vi "Project Lab VIew.vi"() -> ()   [LabVIEW 2026]
uses:
  <vilib>/httpClient/POSTBuffer.vi
  <vilib>/httpClient/LabVIEWHTTPClient.lvlib
panel:
  in  "stop":bool
  out "Supervisory Health Banner":string
  in  "Plant Mode":bool
  out "Web Bridge TX":bool
  out "Live Plant Trend Recorder":cluster{"upper limit":dbl, dbl, dbl}(graph)
  out "CRITICAL PLANT INTERLOCK":bool
  in  "Fan Manual Run":bool
  in  "Valve Override":bool
  out "Fan Active":bool
  out "Valve Open":bool
  in  "Pump Override":bool
  out "Pump Running":bool
  out "Pump Current (A)":dbl(knob) scale=0.0..5.0
  out "12V Bus Voltage (V)":dbl(knob) scale=0.0..20.0
  out "Gas Hazard Level (%)":dbl
  out "Thermometer":dbl(slide) scale=0.0..100.0
  out "Volume (Liters)":dbl
  out "Level (cm)":dbl
  out "Tank Level (cm)":dbl(slide) scale=0.0..100.0
  # "SIMULATION / DIGITAL TWIN"
  # "LIVE HARDWARE (ESP32)"
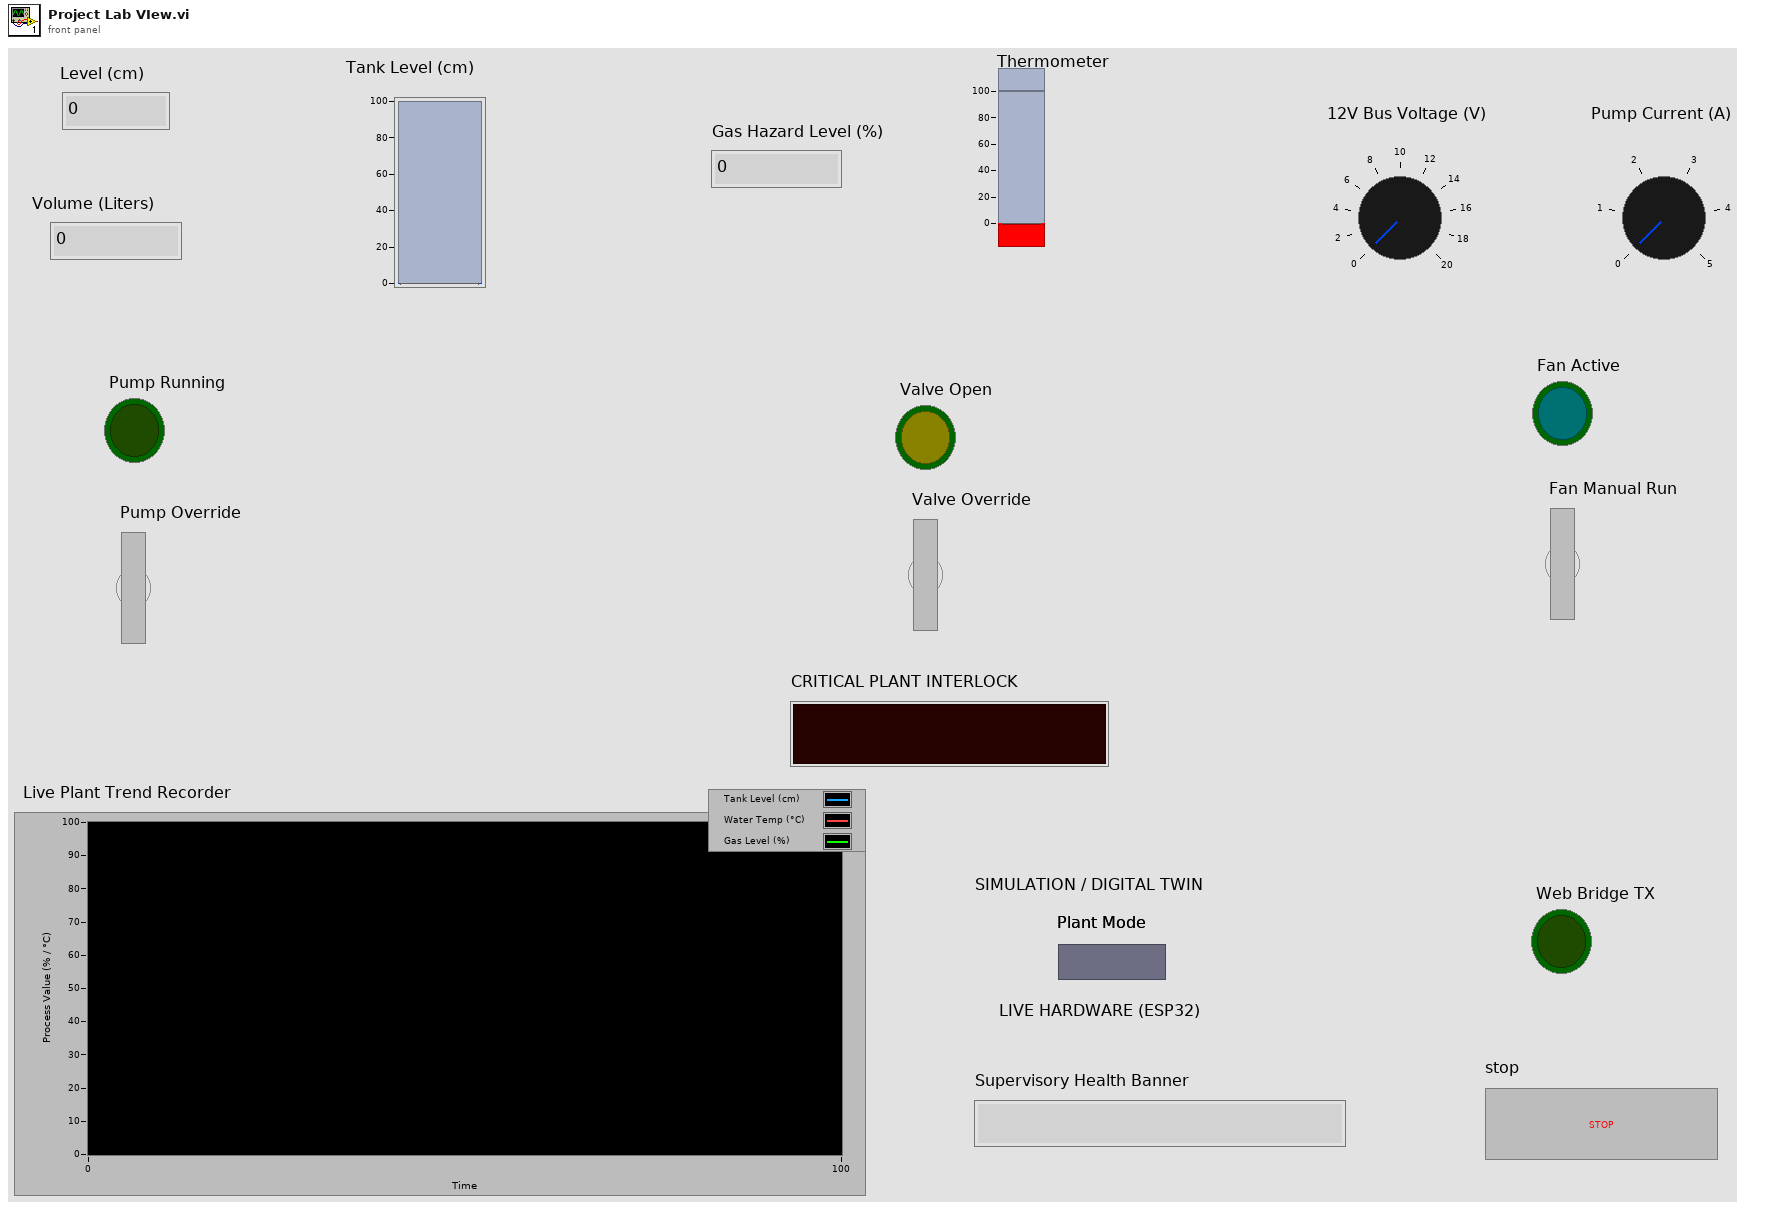
[diagram p1: front panel]
types:
  T1 = cluster{"tank_level":dbl, "temperature":dbl, "gas_ppm":dbl, "current_draw":dbl, "valve_open":bool, "fan_active":bool, "pump_active":bool}
  T2 = cluster{"water_temp_c":dbl, "gas_pct":dbl, "bus_v":dbl, "pump_a":dbl, "pump":dbl, "valve":dbl, "fan":dbl, "alarm":dbl, "level_cm":dbl}
  T3 = cluster{"upper limit":dbl, "water_temp_c":dbl, "gas_pct":dbl}
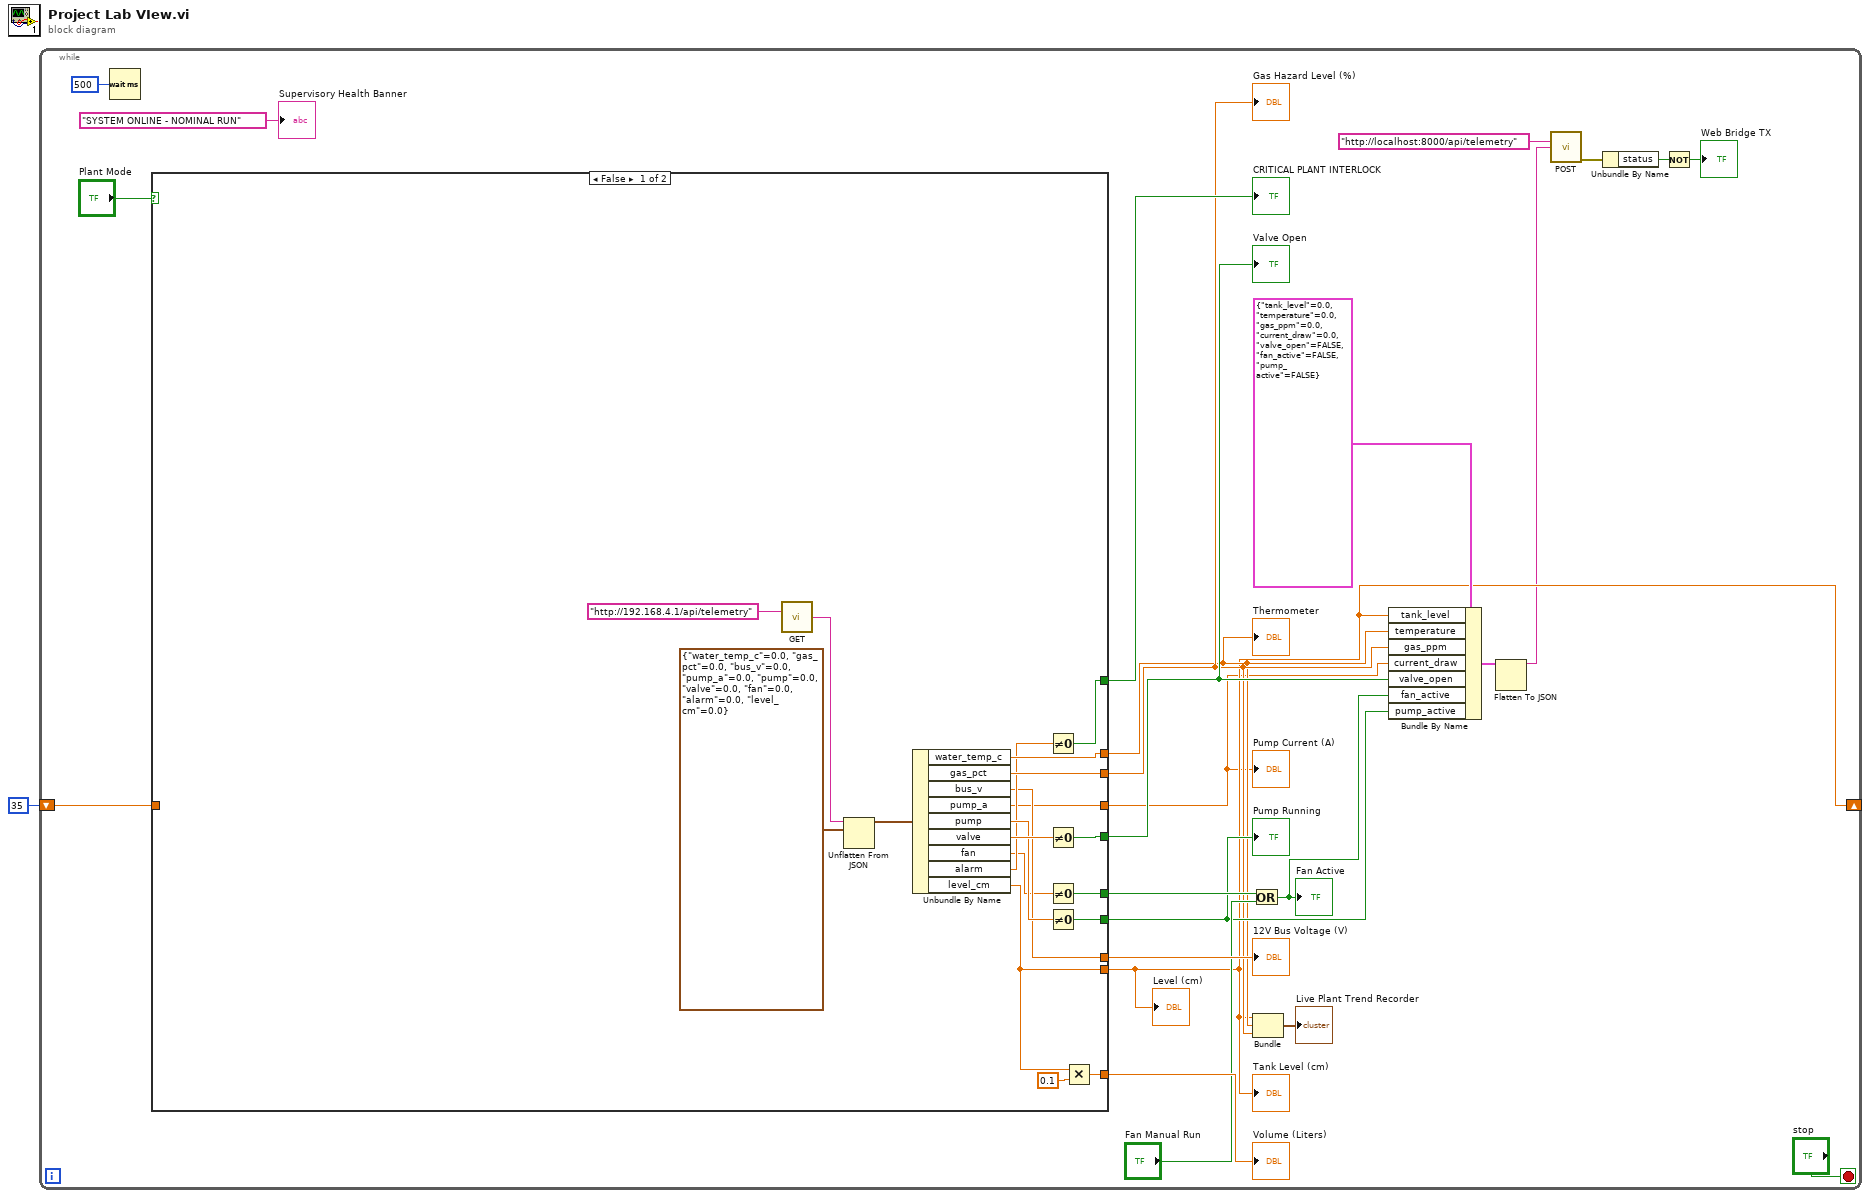
[diagram p0: block diagram]
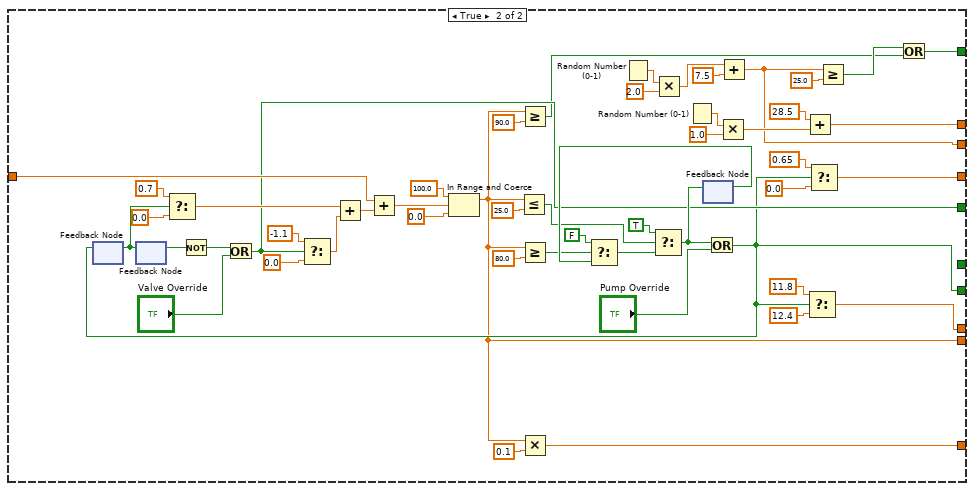
[diagram p2: hidden frame]
diagram:
  n1 = while {
    shift-right: [w9] -> _
    shift-left: u32 35 ("milliseconds to wait") -> [w24]
    stop <- "stop" stop-if-true
    n2 = Wait (ms)(milliseconds to wait=u32 500) -> ()  [unwired: 1 out]
    n3 = case shown="False" "Plant Mode" {
      tunnel: w24 -> [_ w89]
      tunnel: [w39 w52] -> w9
      tunnel: [w40 w71] -> w21
      tunnel: [w42 w66] -> w10
      tunnel: [w38 w50] -> w11
      tunnel: [w31 w58] -> w22
      tunnel: [w30 w55] -> w8
      tunnel: [w33 w53] -> w12
      tunnel: [w34 w54] -> w14
      tunnel: [w32 w46] -> w23
      tunnel: [w27 _] -> w16
      frame False {
        n4 = call <vilib>:"GET.vi"("url"="http://192.168.4.1/api/telemetry") -> ("body"=w29:string)  [unwired: 11 in, 3 out]
        n5 = Unflatten From JSON(JSON string=w29, type and defaults=T2 {"water_temp_c"=0.0, "gas_pct"=0.0, "bus_v"=0.0, "pump_a"=0.0, "pump"=0.0, "valve"=0.0, "fan"=0.0, "alarm"=0.0, "level_cm"=0.0}) -> (value=w43:T2)  [unwired: 5 in, 1 out]
        n6 = Unbundle By Name(w43) -> ("water_temp_c"=w42:dbl, "gas_pct"=w38:dbl, "bus_v"=w31:dbl, "pump_a"=w30:dbl, "pump"=w36:dbl, "valve"=w37:dbl, "fan"=w28:dbl, "alarm"=w35:dbl, "level_cm"=w39:dbl)
        n7 = Not Equal To 0?(x=w35) -> (x != 0?=w32:bool)
        n8 = Not Equal To 0?(x=w37) -> (x != 0?=w34:bool)
        n9 = Not Equal To 0?(x=w28) -> (x != 0?=w27:bool)
        n10 = Not Equal To 0?(x=w36) -> (x != 0?=w33:bool)
        n11 = Multiply(x=w39, y=0.1) -> (x*y=w40:dbl)
      }
      frame True {
        n12 = feedback #1() -> (w61:bool)  [unwired: 1 in]
        n13 = feedback-in #2(w61) -> ()
        n14 = feedback #2() -> (w73:bool)  [unwired: 1 in]
        n15 = Select(t=0.7, s=w61, f=0.0) -> (s? t:f=w92:dbl)
        n16 = Not(x=w73) -> (.not. x?=w77:bool)
        n17 = Or(x=w77, y="Valve Override") -> (x .or. y?=w54:bool)
        n18 = Select(t=-1.1, s=w54, f=0.0) -> (s? t:f=w91:dbl)
        n19 = Add(x=w92, y=w91) -> (x+y=w90:dbl)
        n20 = Add(x=w89, y=w90) -> (x+y=w86:dbl)
        n21 = In Range and Coerce(upper limit=100.0, x=w86, lower limit=0.0) -> (coerced(x)=w52:dbl)  [unwired: 1 out]
        n22 = Less Or Equal?(x=w52, y=25.0) -> (x <= y?=w75:bool)
        n23 = Greater Or Equal?(x=w52, y=90.0) -> (x >= y?=w47:bool)
        n24 = Greater Or Equal?(x=w52, y=80.0) -> (x >= y?=w74:bool)
        n25 = Multiply(x=w52, y=0.1) -> (x*y=w71:dbl)
        n26 = Random Number (0-1)() -> (number: 0 to 1=w65:dbl)
        n27 = Multiply(x=w65, y=2.0) -> (x*y=w63:dbl)
        n28 = Random Number (0-1)() -> (number: 0 to 1=w70:dbl)
        n29 = feedback #3() -> (w80:bool)  [unwired: 1 in]
        n30 = Select(t=FALSE, s=w74, f=w80) -> (s? t:f=w81:bool)
        n31 = Select(t=TRUE, s=w75, f=w81) -> (s? t:f=w78:bool)
        n32 = feedback-in #3(w78) -> ()
        n33 = Or(x=w78, y="Pump Override") -> (x .or. y?=w53:bool)
        n34 = feedback-in #1(w53) -> ()
        n35 = Multiply(x=w70, y=1.0) -> (x*y=w68:dbl)
        n36 = Add(x=w63, y=7.5) -> (x+y=w50:dbl)
        n37 = Add(x=28.5, y=w68) -> (x+y=w66:dbl)
        n38 = Select(t=11.8, s=w53, f=12.4) -> (s? t:f=w58:dbl)
        n39 = Select(t=0.65, s=w53, f=0.0) -> (s? t:f=w55:dbl)
        n40 = Greater Or Equal?(x=w50, y=25.0) -> (x >= y?=w48:bool)
        n41 = Or(x=w48, y=w47) -> (x .or. y?=w46:bool)
      }
    }
    "CRITICAL PLANT INTERLOCK" <- w23
    "Thermometer" <- w10
    "Volume (Liters)" <- w21
    "Gas Hazard Level (%)" <- w11
    "Valve Open" <- w14
    "Pump Current (A)" <- w8
    "Pump Running" <- w12
    "12V Bus Voltage (V)" <- w22
    "Tank Level (cm)" <- w9
    "Level (cm)" <- w9
    n42 = Or(x=w16, y="Fan Manual Run") -> (x .or. y?=w13:bool)
    "Fan Active" <- w13
    n43 = Bundle("upper limit"=w9, "water_temp_c"=w10, "gas_pct"=w11) -> (→"Live Plant Trend Recorder":T3)  [unwired: 1 in]
    n44 = Bundle By Name(cluster=T1 {"tank_level"=0.0, "temperature"=0.0, "gas_ppm"=0.0, "current_draw"=0.0, "valve_open"=FALSE, "fan_active"=FALSE, "pump_active"=FALSE}, "tank_level"=w9, "temperature"=w10, "gas_ppm"=w11, "current_draw"=w8, "valve_open"=w14, "fan_active"=w13, "pump_active"=w12) -> (w7:T1)
    n45 = Flatten To JSON(anything=w7) -> (JSON string=w5:string)  [unwired: 2 in, 1 out]
    n46 = call-poly <vilib>:"POST.vi"("url"="http://localhost:8000/api/telemetry", "buffer"=w5) -> ("error out"=w4:errorcluster)  [unwired: 10 in, 3 out]
    n47 = Unbundle By Name(w4) -> ("status"=w3:bool)
    n48 = Not(x=w3) -> (.not. x?=→"Web Bridge TX":bool)
    "Supervisory Health Banner" <- "SYSTEM ONLINE - NOMINAL RUN" ("Supervisory Health Banner")
  }
